vi "AlliGator Source Image Event Registration.vi"(8 "error in (no error)":errorcluster) -> (0 "error out":errorcluster, 2 "Time Point Slide Event Registration":refnum<event-registration>, 3 "Source Image Display Event Registration":refnum<event-registration>)   [LabVIEW 2021, in "AlliGator GUI.lvlib"]
uses:
  GUI/AlliGator GUI.lvlib
panel:
  # "see the License on the block diagram (Ctrl+E or Window:Show Block Diagram)"
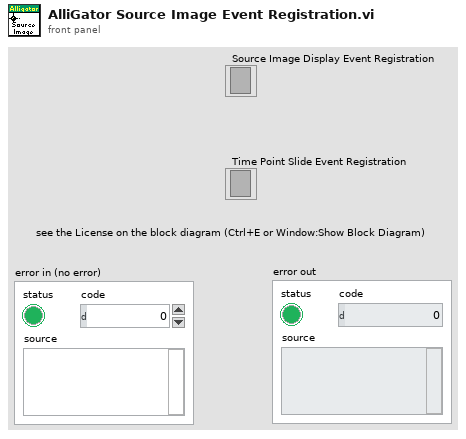
[diagram p1: front panel]
types:
  T1 = typedef "AlliGator GUI.lvlib/AlliGator Dataset Ctrl Refnums.ctl" = cluster{"Current Data":refnum<vi>, "Gate Image Slide":refnum<vi>, "Time Point Slide":refnum<vi>, "Current Time Stamp":refnum<vi>, "Save Image":refnum<vi>, "Displayed Image":refnum<vi>, "Phasor Overlay Color":refnum<vi>, "Image Color Scale":refnum<vi>, "Use ROI as Search Area":refnum<vi>, "Source Image ROI Color":refnum<vi>, "True Pixel Value":refnum<vi>, "Source Image Display":refnum<vi>, "CPU":refnum<vi>}
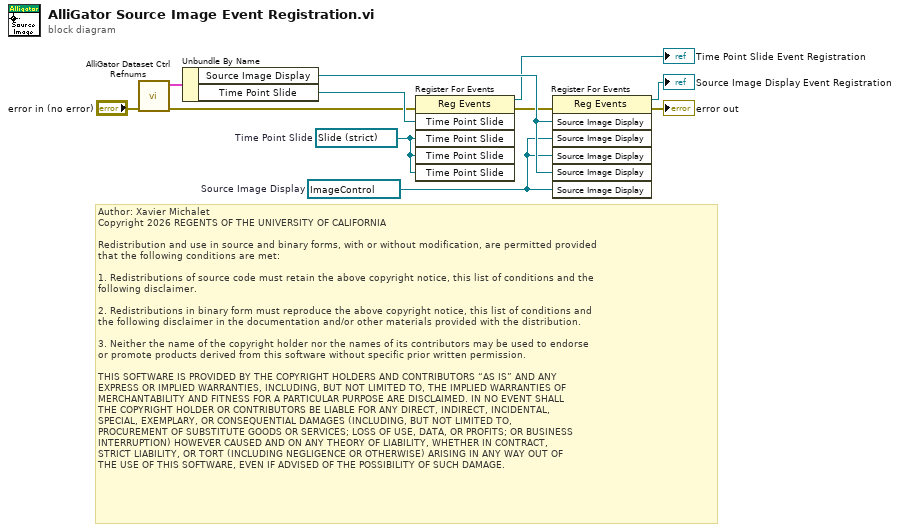
[diagram p0: block diagram]
diagram:
  w7 = refnum<vi> refnum  # Time Point Slide
  w3 = refnum<vi> refnum  # Source Image Display
  # "Author: Xavier Michalet\nCopyright 2026 REGENTS OF THE UNIVERSITY OF CALIFORNIA\n\nRedistribution and use in source and binary forms, with or without modification, are permitted provided\nthat the following conditions are met:\n\n1. Redistributions of source code must retain the above copyright notice, this list of conditions and the\nfollowing disclaimer.\n\n2. Redistributions in binary form must reproduce the above copyright notice, this list of conditions and\nthe following disclaimer in the documentation and/or other materials provided with the distribution.\n\n3. Neither the name of the copyright holder nor the names of its contributors may be used to endorse \nor promote products derived from this software without specific prior written permission.\n\nTHIS SOFTWARE IS PROVIDED BY THE COPYRIGHT HOLDERS AND CONTRIBUTORS “AS IS” AND ANY \nEXPRESS OR IMPLIED WARRANTIES, INCLUDING, BUT NOT LIMITED TO, THE IMPLIED WARRANTIES OF\nMERCHANTABILITY AND FITNESS FOR A PARTICULAR PURPOSE ARE DISCLAIMED. IN NO EVENT SHALL\nTHE COPYRIGHT HOLDER OR CONTRIBUTORS BE LIABLE FOR ANY DIRECT, INDIRECT, INCIDENTAL, \nSPECIAL, EXEMPLARY, OR CONSEQUENTIAL DAMAGES (INCLUDING, BUT NOT LIMITED TO, \nPROCUREMENT OF SUBSTITUTE GOODS OR SERVICES; LOSS OF USE, DATA, OR PROFITS; OR BUSINESS\nINTERRUPTION) HOWEVER CAUSED AND ON ANY THEORY OF LIABILITY, WHETHER IN CONTRACT, \nSTRICT LIABILITY, OR TORT (INCLUDING NEGLIGENCE OR OTHERWISE) ARISING IN ANY WAY OUT OF\nTHE USE OF THIS SOFTWARE, EVEN IF ADVISED OF THE POSSIBILITY OF SUCH DAMAGE."
  n1 = call "AlliGator Dataset Ctrl Refnums.vi"("error in (no error)"="error in (no error)") -> ("error out"=w2:errorcluster, "Dataset Control References"=w10:T1)  [unwired: 9 in]
  n2 = Unbundle By Name(w10) -> ("Source Image Display"=w8:refnum<vi>, "Time Point Slide"=w9:refnum<vi>)
  n3 = register-events(error in=w2, w9, w7, w7, w7) -> (reference out=→"Time Point Slide Event Registration":refnum<event-registration>, error out=w1:errorcluster)  [unwired: 1 in]
  n4 = register-events(error in=w1, w8, w3, w3, w8, w3) -> (reference out=→"Source Image Display Event Registration":refnum<event-registration>, error out=→"error out":errorcluster)  [unwired: 1 in]
